vi "Test.vi"() -> ()   [LabVIEW 2019]
uses:
  <vilib>/Skyline/AssetManagement/Start Utilization (All).vi
  <vilib>/Skyline/AssetManagement/Start Utilization (Single).vi
  <vilib>/Skyline/AssetManagement/NI SystemLink Asset Utilization.lvclass
panel:
  in  "Initial Capacity  (mAh) in":dbl=2500.0 format="%#_13g"
  out "Numeric":i32
  out "Waveform Graph":dbl[](graph)
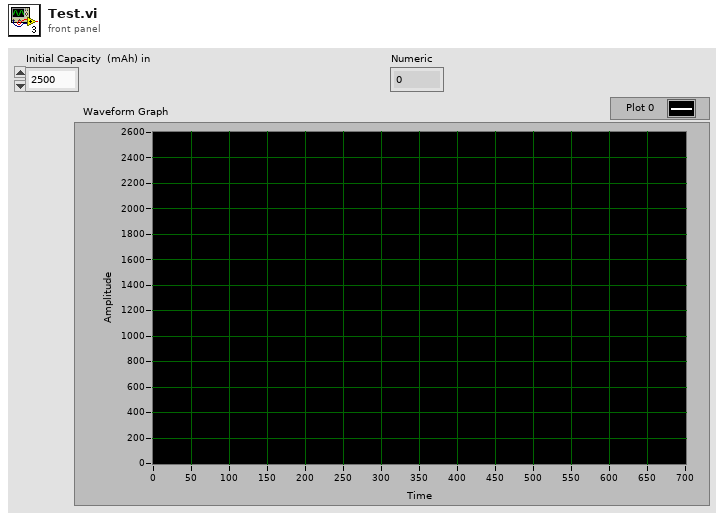
[diagram p1: front panel]
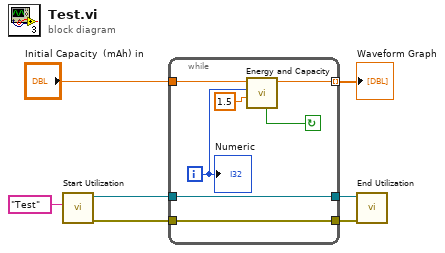
[diagram p0: block diagram]
diagram:
  n1 = call-poly <vilib>:"Start Utilization.vi"("utilization category"="Test") -> ("error out"=w2:errorcluster, "asset utilization"=w4:refnum<class "NI SystemLink Asset Utilization.lvclass">)  [unwired: 9 in]
  n2 = while {
    tunnel: [w14] -> w7 mode=indexing
    tunnel: "Initial Capacity  (mAh) in" -> [w10]
    tunnel: [w9] -> w5
    tunnel: w4 -> [w9]
    tunnel: [w8] -> w3
    tunnel: w2 -> [w8]
    i -> [w13]
    stop <- w11 continue-if-true
    n3 = call "Energy and Capacity.vi"("Voltage"=1.5, "Cycle"=w13, "Initial Capacity  (mAh) in"=w10) -> ("Capacity  (mAh)"=w14:dbl, "Pass"=w11:bool)  [unwired: 4 in, 3 out]
    "Numeric" <- w13
  }
  "Waveform Graph" <- w7
  n4 = call <vilib>:"End Utilization.vi"("error in (no error)"=w3, "asset utilization"=w5) -> ()  [unwired: 9 in, 1 out]
